vi "Public Key Data Authentication.vi"(4 "Key Files":cluster{"Private":path, "Public":path}={"Private"=path "", "Public"=path ""}, 5 "Username":string, 6 "Passphrase":string, 7 "Address":string, 8 "Error In":errorcluster) -> (0 "Error Out":errorcluster)   [LabVIEW 2018, in "Tests.lvlib" / "Session.lvlib"]
uses:
  Session.lvlib
  Support/SSH Key Types.ctl
  Support/Secret Types.ctl
  Support/Select Key File.vi
  src/Toolkit/Session/Support/Create from SSH.vi
  <vilib>/Utility/sysdir.llb/Get System Directory.vi
  src/Toolkit/Session/Support/Public Key Memory Authentication.vi
  src/Toolkit/Session/Support/Destroy to SSH.vi
  <vilib>/addons/_JKI Toolkits/Caraya/classes/Test/Test.lvclass
  src/Toolkit/SSH/SSH.lvclass
  src/Toolkit/Session/Session.lvclass
  <vilib>/addons/_JKI Toolkits/Caraya/classes/Assert/Assert.lvclass
  Tests.lvlib
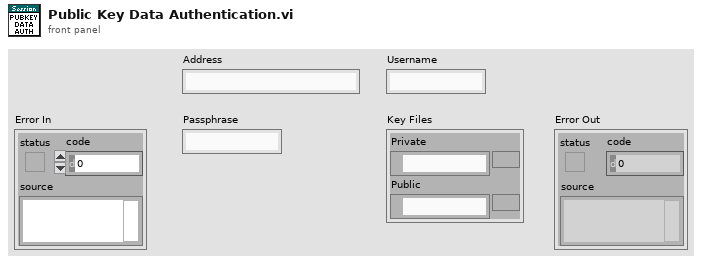
[diagram p1: front panel]
types:
  T1 = typedef "Tests.lvlib/SSH Key Types.ctl" = enum16{"Private", "Public"}
  T2 = typedef "Tests.lvlib/Secret Types.ctl" = enum16{"Passphrase", "Password"}
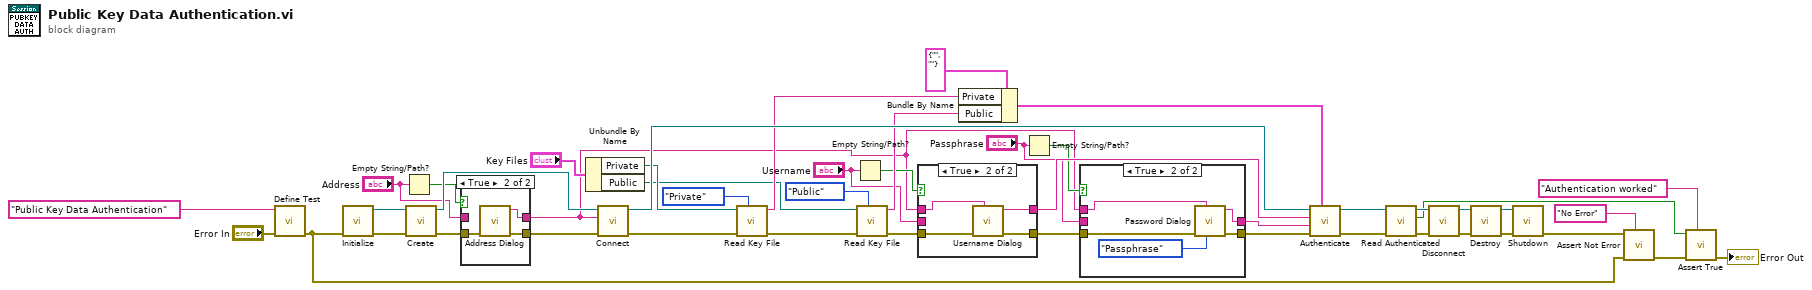
[diagram p0: block diagram]
diagram:
  n1 = call <vilib>:"Define Test.vi"("error in (no error)"="Error In", "Label (VI Title)"="Public Key Data Authentication") -> ("error out"=w38:errorcluster)  [unwired: 9 in]
  n2 = call "Initialize.vi"("Error In"=w38) -> ("Error Out"=w44:errorcluster, "SSH"=w43:refnum<class "SSH.lvclass">)  [unwired: 9 in]
  n3 = Empty String/Path?(string/path="Address") -> (empty?=w22:bool)
  n4 = call-poly "Create.vi"("Error In"=w44, "SSH"=w43) -> ("Error Out"=w21:errorcluster, "Sesssion"=w36:refnum<class "Session.lvclass">)  [unwired: 8 in]
  n5 = case shown="True" w22 {
    tunnel: w21 -> [w47 w51]
    tunnel: [w47 w50] -> w20
    tunnel: [w48 w49] -> w1
    tunnel: "Address" -> [w48 _]
    frame False {
    }
    frame True {
      n6 = call "Address Dialog.vi"("Error In"=w51) -> ("Error Out"=w50:errorcluster, "Address Out"=w49:string)  [unwired: 9 in]
    }
  }
  n7 = Unbundle By Name("Key Files") -> ("Private"=w3:path, "Public"=w2:path)
  n8 = call "Connect.vi"("Error In"=w20, "Address"=w1, "Session In"=w36) -> ("Error Out"=w18:errorcluster, "Sesssion Out"=w33:refnum<class "Session.lvclass">)  [unwired: 7 in]
  n9 = call "Read Key File.vi"("Key Type"=SSH_Key_Types."Private", "Error In"=w18, "Key File"=w3) -> ("Error Out"=w15:errorcluster, "Key Data"=w23:string)  [unwired: 7 in]
  n10 = Empty String/Path?(string/path="Username") -> (empty?=w13:bool)
  n11 = call "Read Key File.vi"("Key Type"=SSH_Key_Types."Public", "Error In"=w15, "Key File"=w2) -> ("Error Out"=w12:errorcluster, "Key Data"=w14:string)  [unwired: 7 in]
  n12 = case shown="True" w13 {
    tunnel: w12 -> [w52 w57]
    tunnel: [w53 w56] -> w11
    tunnel: [w52 w55] -> w9
    tunnel: "Username" -> [w53 _]
    tunnel: w1 -> [_ w54]
    frame False {
    }
    frame True {
      n13 = call "Username Dialog.vi"("Address"=w54, "Error In"=w57) -> ("Error Out"=w55:errorcluster, "Username Out"=w56:string)  [unwired: 8 in]
    }
  }
  n14 = Bundle By Name(cluster=cluster{"Private":string, "Public":string} {"Private"="", "Public"=""} ("Keys"), "Private"=w23, "Public"=w14) -> (w24:cluster{"Private":string, "Public":string})
  n15 = Empty String/Path?(string/path="Passphrase") -> (empty?=w5:bool)
  n16 = case shown="True" w5 {
    tunnel: w9 -> [w58 w64]
    tunnel: [w58 w63] -> w8
    tunnel: [w59 w62] -> w7
    tunnel: "Passphrase" -> [w59 _]
    tunnel: w1 -> [_ w61]
    frame False {
    }
    frame True {
      n17 = call "Password Dialog.vi"("Secret Type"=Secret_Types."Passphrase", "Address"=w61, "Error In"=w64) -> ("Error Out"=w63:errorcluster, "Password Out"=w62:string)  [unwired: 7 in]
    }
  }
  n18 = call-poly "Authenticate.vi"("Keys"=w24, "Error In"=w8, "Passphrase"=w7, "Username"=w11, "Session In"=w33) -> ("Error Out"=w31:errorcluster, "Sesssion Out"=w32:refnum<class "Session.lvclass">)  [unwired: 5 in]
  n19 = call "Read Authenticated.vi"("Error In"=w31, "Session In"=w32) -> ("Error Out"=w30:errorcluster, "Authenticated"=w27:bool, "Sesssion Out"=w29:refnum<class "Session.lvclass">)  [unwired: 7 in]
  n20 = call "Disconnect.vi"("Error In"=w30, "Session In"=w29) -> ("Error Out"=w34:errorcluster, "Sesssion Out"=w35:refnum<class "Session.lvclass">)  [unwired: 8 in]
  n21 = call-poly "Destroy.vi"("Error In"=w34, "Session"=w35) -> ("Error Out"=w41:errorcluster, "SSH"=w42:refnum<class "SSH.lvclass">)  [unwired: 8 in]
  n22 = call "Shutdown.vi"("Error In"=w41, "SSH"=w42) -> ("Error Out"=w40:errorcluster)  [unwired: 9 in]
  n23 = call <vilib>:"Assert Not Error.vi"("Label"="No Error", "error in (no error)"=w38, "Not Error?"=w40) -> ("error out"=w37:errorcluster)  [unwired: 8 in]
  n24 = call <vilib>:"Assert True.vi"("Label"="Authentication worked", "error in (no error)"=w37, "True?"=w27) -> ("error out"=→"Error Out":errorcluster)  [unwired: 8 in]
